vi "gRPC Server.vi"(8 "error in (no error)":errorcluster, 11 "CIFPlugin in":refnum<class "CAN_Writer_CANsub_Plugin.lvclass">) -> (0 "error out":errorcluster, 3 "CIFPlugin out":refnum<class "CAN_Writer_CANsub_Plugin.lvclass">)   [LabVIEW 2021, in "CAN_Writer_CANsub_Plugin.lvclass"]
uses:
  CAN_Writer_CANsub_Plugin.lvclass
  CAN_Writer_CANsub_Plugin.lvclass/CAN_Writer_CANsub_Plugin.ctl
  <vilib>/CIF Foundation/CIF Core/CIFCore/Class/CIFCorePlugin.lvclass
  Grpc/CanWriterCansub_server/RPC Messages/cif_common_Status.ctl
  Grpc/CanWriterCansub_server/CanWriterCansub_server.lvlib
  Grpc/CanWriterCansub_server/RPC Messages/cif_can_writer_cansub_Statistics.ctl
  Grpc/CanWriterCansub_server/RPC Service/CanWriterCansub/CanWriterCansub.lvclass
  <vilib>/CIF Foundation/CIF XNET CAN RW/XNET CAN RW.lvclass
  <vilib>/xnet/xnet.llb/XNET Blink Modifier.ctl
  Common/CAN_Writer_CANsub_Common.lvlib
  Common/Typedef/Errors.ctl
  Grpc/CanWriterCansub_server/RPC Messages/cif_can_writer_cansub_CommState.ctl
  Grpc/CanWriterCansub_server/RPC Messages/cif_can_writer_cansub_LastError.ctl
  Grpc/CanWriterCansub_server/RPC Messages/cif_can_writer_cansub_GetCANStatusResponse.ctl
  Grpc/CanWriterCansub_server/RPC Messages/cif_can_writer_cansub_CansubDevice.ctl
  Grpc/CanWriterCansub_server/RPC Messages/cif_can_writer_cansub_CansubDevices.ctl
  C:/Program Files/National Instruments/LabVIEW 2021/vi.lib/CIF Foundation/CIF Core/CIFCore/Class/CIFCorePlugin.lvclass
  D:/dev/Plugins/CAN_Writer_CANsub/Class/CAN_Writer_CANsub_Plugin.lvclass
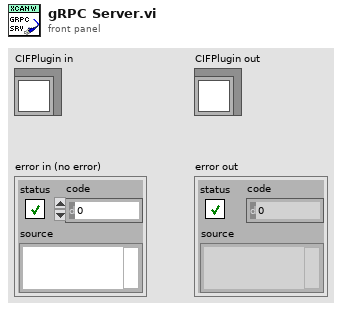
[diagram p1: front panel]
types:
  T1 = typedef "CanWriterCansub_server.lvlib/cif_can_writer_cansub_CansubDevices.ctl" = cluster{"devices":T2[]}
  T2 = typedef "CanWriterCansub_server.lvlib/cif_can_writer_cansub_CansubDevice.ctl" = cluster{"interface":string, "slot":u32, "device_id":string}
  T3 = typedef "CanWriterCansub_server.lvlib/cif_can_writer_cansub_GetCANStatusResponse.ctl" = cluster{"comm_state":T4, "last_error":T5, "rx_error_ctr":u32, "tx_error_crt":u32}
  T4 = typedef "CanWriterCansub_server.lvlib/cif_can_writer_cansub_CommState.ctl" = enum32{"COMMSTATE_ERROR_ACTIVE", "COMMSTATE_ERROR_PASSIVE", "COMMSTATE_BUS_OFF"}
  T5 = typedef "CanWriterCansub_server.lvlib/cif_can_writer_cansub_LastError.ctl" = enum32{"LASTERROR_NONE", "LASTERROR_STUFF", "LASTERROR_FORM", "LASTERROR_ACK", "LASTERROR_BIT1", "LASTERROR_BIT0", "LASTERROR_CRC", "LASTERROR_UNKNOWN"}
  T6 = typedef "CanWriterCansub_server.lvlib/cif_common_Status.ctl" = cluster{"code":i32, "message":string}
  T7 = typedef "CAN_Writer_CANsub_Common.lvlib/Errors.ctl" = enum16{"Invalid Interface"}
  T8 = typedef "XNET CAN RW.lvclass/XNET Devices.ctl" = cluster{"ID":string, "Slot":u32, "Interfaces":string[]}
  T9 = typedef "grpc-lvsupport-release.lvlib/grpcId.ctl" = u64
  T10 = typedef "CanWriterCansub_server.lvlib/cif_can_writer_cansub_CanMessage.ctl" = cluster{"can_message":u8[]}
  T11 = typedef "CanWriterCansub_server.lvlib/cif_can_writer_cansub_RefreshDevices.ctl" = cluster{"refresh_device_list":bool}
  T12 = typedef "CanWriterCansub_server.lvlib/cif_can_writer_cansub_Statistics.ctl" = cluster{"iterations":u64, "fifo_read_timeouts":u64, "write_frames":u64, "filtered_frames":u64, "fifo_drops":u64, "ack_errors":u64}
  T13 = typedef "CAN_RW_CORE.lvclass/Communication State.ctl" = enum16{"Error Active", "Error Passive", "Bus Off"}
  T14 = typedef "CAN_RW_CORE.lvclass/Last Error.ctl" = enum16{"None", "Stuff", "Form", "Ack", "Bit1", "Bit0", "CRC", "Unknown"}
  T15 = typedef "XNET Blink Modifier.ctl" = u32
  T16 = typedef "CanWriterCansub_server.lvlib/cif_can_writer_cansub_InterfaceBlink.ctl" = cluster{"blink":bool}
  T17 = typedef "CAN_Writer_CANsub_Common.lvlib/Configuration.ctl" = cluster{"Common":T18, "TX Interface":string, "Port Configuration":T20, "Filter":T23, "Wake Offset (us)":i64, "One Shot":bool}
  T18 = typedef "CIFCoreCommon.lvlib/Common Plugin Configuration.ctl" = cluster{"Period (s)":dbl, "Offset (us)":i32, "Priority":i32, "Processor":i32, "External Clock":T19}
  T19 = typedef "CIFCoreCommon.lvlib/External Clock Config.ctl" = cluster{"ClockID":u8, "Clock Name":string, "Publish Clock":bool, "Convert Data Timestamps":bool, "Plugin Timing Source":bool}
  T20 = typedef "CAN_RW_CORE.lvclass/CAN Port Configuration.ctl" = cluster{"Mode":T21, "Baud Rate":u64, "Temination On":bool, "Subordinate":bool, "Echo TX":bool, "FD Config":T22}
  T21 = typedef "CAN_RW_CORE.lvclass/CAN Mode.ctl" = enum16{"CAN 2.0", "CAN FD"}
  T22 = typedef "CAN_RW_CORE.lvclass/FD Config.ctl" = cluster{"FD Baud Rate":u64, "ISO Mode":bool, "BRS Enabled":bool}
  T23 = typedef "CAN_RW_CORE.lvclass/CAN Filter.ctl" = cluster{"Allow List (ID)":u32[], "Deny List (ID)":u32[]}
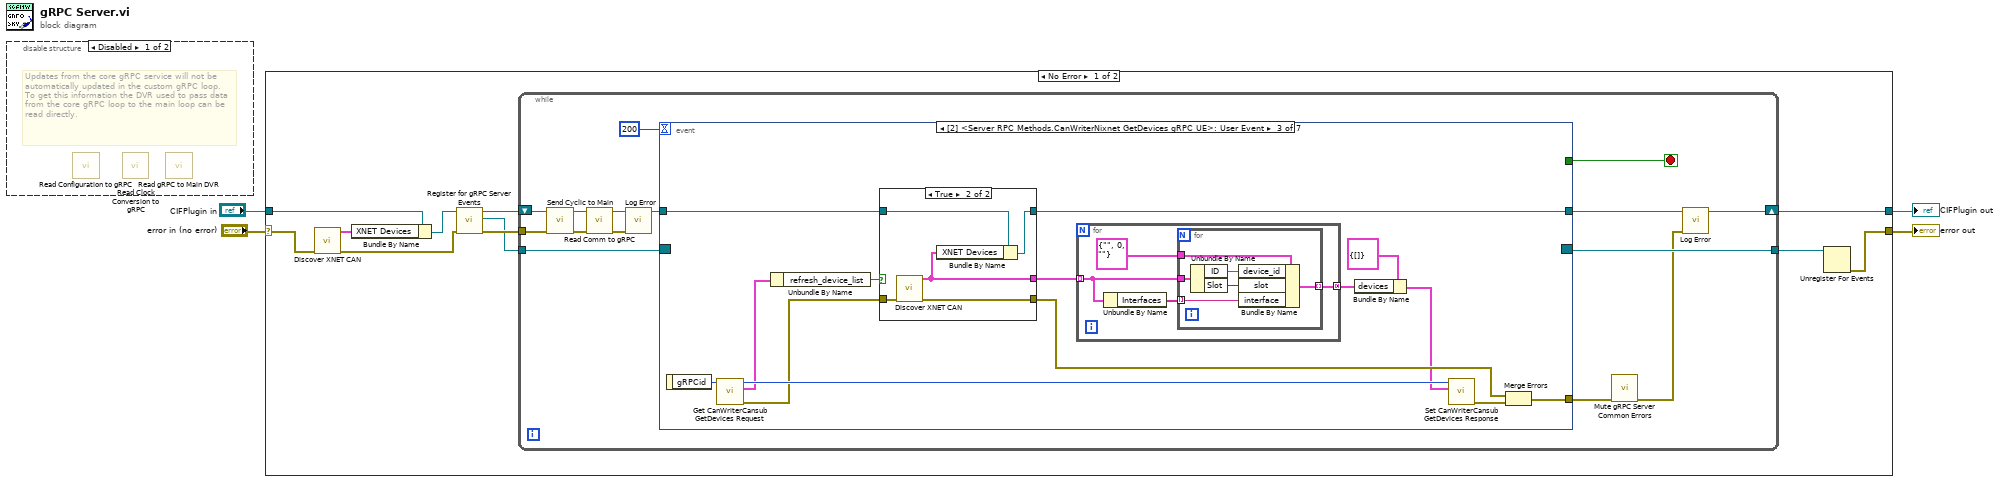
[diagram p0: block diagram]
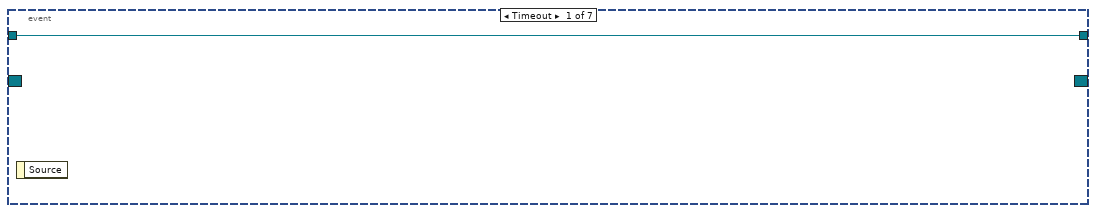
[diagram p3: hidden frame]
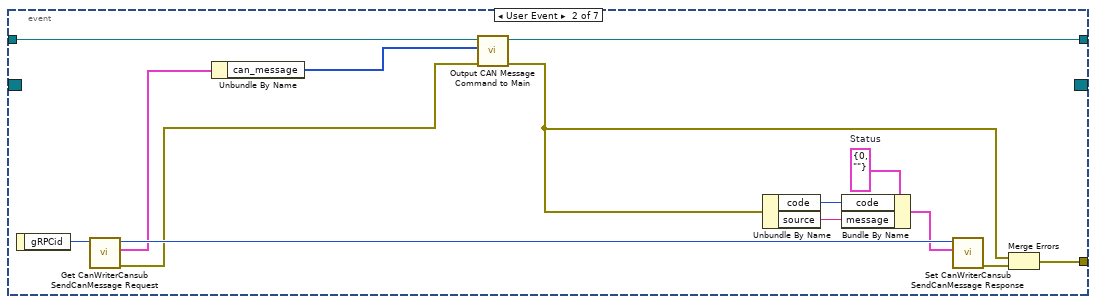
[diagram p4: hidden frame]
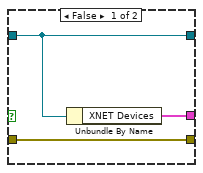
[diagram p5: hidden frame]
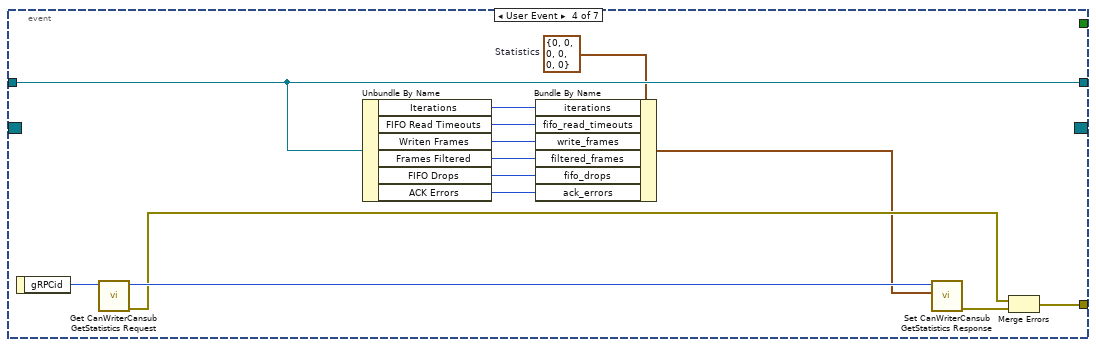
[diagram p6: hidden frame]
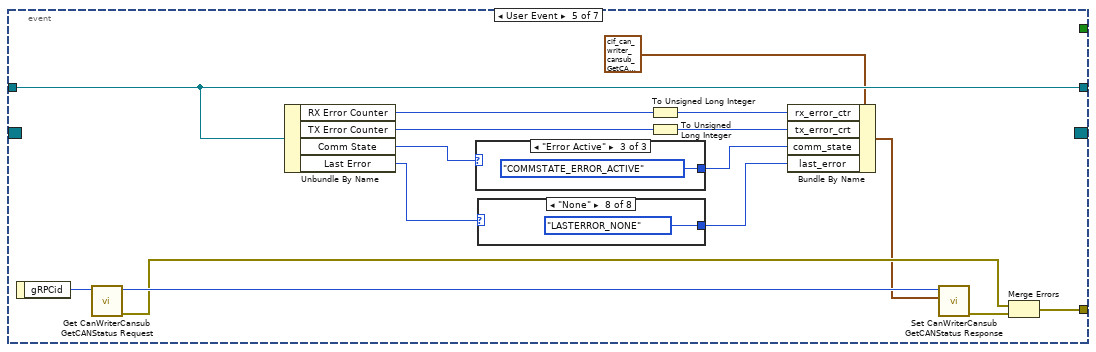
[diagram p7: hidden frame]
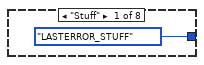
[diagram p8: hidden frame]
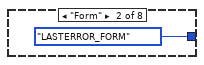
[diagram p9: hidden frame]
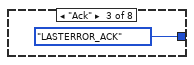
[diagram p10: hidden frame]
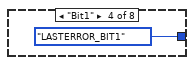
[diagram p11: hidden frame]
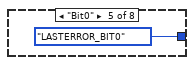
[diagram p12: hidden frame]
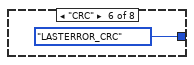
[diagram p13: hidden frame]
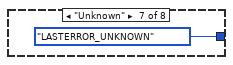
[diagram p14: hidden frame]
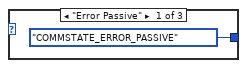
[diagram p15: hidden frame]
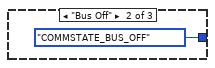
[diagram p16: hidden frame]
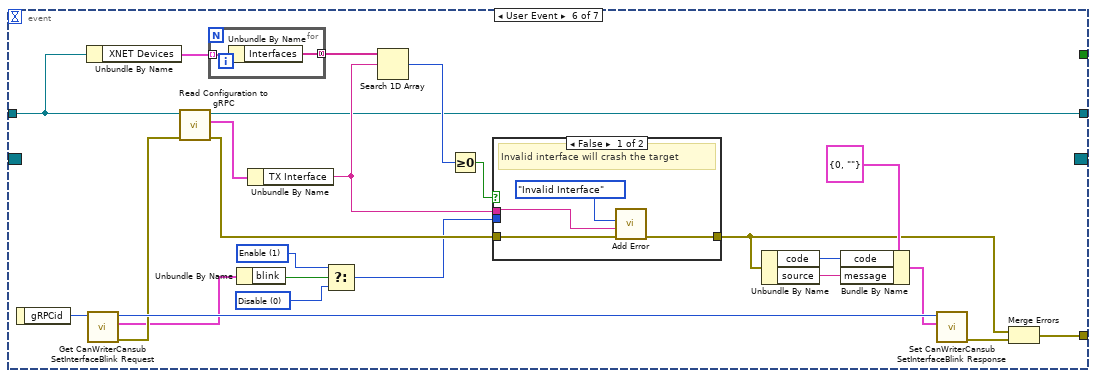
[diagram p17: hidden frame]
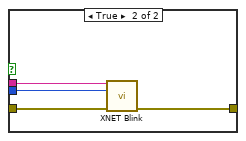
[diagram p18: hidden frame]
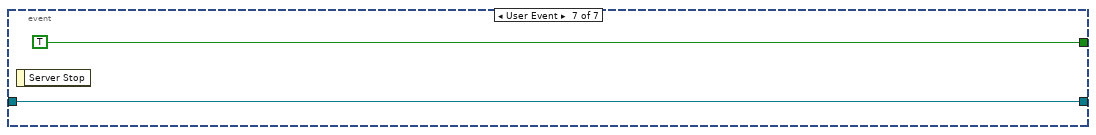
[diagram p19: hidden frame]
diagram:
  n1 = disable-structure shown="Disabled" {
    frame Disabled {
      # "Updates from the core gRPC service will not be automatically updated in the custom gRPC loop.  To get this information the DVR used to pass data from the core gRPC loop to the main loop can be read directly."
      n2 = call "Read Configuration to gRPC.vi"() -> ()  [unwired: 9 in, 3 out]
      n3 = call <vilib>:"Read Clock Conversion to gRPC.vi"() -> ()  [unwired: 9 in, 3 out]
      n4 = call <vilib>:"Read gRPC to Main DVR.vi"() -> ()  [unwired: 9 in, 3 out]
    }
    frame Enabled {
    }
  }
  n5 = case shown="No Error" "error in (no error)" {
    selector: "error in (no error)" -> [w6 w155]
    tunnel: "CIFPlugin in" -> [w9 w156]
    tunnel: [w14 w156] -> w3
    tunnel: [w11 w155] -> w4
    frame No Error {
      n6 = call <vilib>:"Discover XNET CAN.vi"("error in (no error)"=w6) -> ("error out"=w5:errorcluster, "XNET Devices"=w7:T8[])  [unwired: 9 in]
      n7 = Bundle By Name(cluster=w9, "XNET Devices"=w7) -> (w8:refnum<class "CAN_Writer_CANsub_Plugin.lvclass">)
      n8 = call "Register for gRPC Server Events.vi"("error in (no error)"=w5, "CIFPlugin in"=w8) -> ("error out"=w13:errorcluster, "Event Registration Refnum"=w10:refnum<event-registration>, "CIFPlugin out"=w12:refnum<class "CAN_Writer_CANsub_Plugin.lvclass">)  [unwired: 7 in]
      n9 = while {
        tunnel: w10 -> [w18]
        tunnel: w13 -> [w23]
        tunnel: [w28] -> w15
        shift-right: [w26] -> w14
        shift-left: w12 -> [w24]
        stop <- w29 stop-if-true
        n10 = call "Send Cyclic to Main.vi"("error in (no error)"=w23, "CIFPlugin in"=w24) -> ("error out"=w21:errorcluster, "CIFPlugin out"=w22:refnum<class "CAN_Writer_CANsub_Plugin.lvclass">)  [unwired: 8 in]
        n11 = call "Read Comm to gRPC.vi"("error in (no error)"=w21, "CIFPlugin in"=w22) -> ("error out"=w19:errorcluster, "CIFPlugin out"=w20:refnum<class "CAN_Writer_CANsub_Plugin.lvclass">)  [unwired: 8 in]
        n12 = call <vilib>:"Log Error.vi"("error in (no error)"=w19, "CIFCorePlugin in"=w20) -> ("CIFCorePlugin out"=w25:refnum<class "CAN_Writer_CANsub_Plugin.lvclass">)  [unwired: 8 in, 1 out]
        n13 = event shown="[2] <Server RPC Methods.CanWriterNixnet GetDevices gRPC UE>: User Event" {
          selector: w18 -> [_ _ _ _ _ _ _]
          dyn-events: [_ _ _ _ _ _ _] -> w28
          timeout: 200 -> [_ _ _ _ _ _ _]
          tunnel: w25 -> [w31 w36 w50 w90 w106 w119 w153]
          tunnel: [_ w43 w59 w91 w107 w142 _] -> w17
          tunnel: [w31 w32 w49 w90 w106 w125 w153] -> w27
          tunnel: [_ _ _ _ _ _ TRUE] -> w29
          event Timeout {
            n14 = event-data() -> ()  [unwired: 1 in, 1 out]
          }
          event User Event {
            w42 = T6 {"code"=0, "message"=""}  # Status
            n15 = event-data() -> ("gRPCid"=w40:T9)  [unwired: 1 in]
            n16 = call "Get CanWriterCansub SendCanMessage Request.vi"("gRPCid"=w40) -> ("error out"=w34:errorcluster, "Message Data"=w38:T10, "gRPCid out"=w41:T9)  [unwired: 8 in]
            n17 = Unbundle By Name(w38) -> ("can_message"=w35:u8[])
            n18 = call "Output CAN Message Command to Main.vi"("error in (no error)"=w34, "Output Message"=w35, "CIFPlugin in"=w36) -> ("error out"=w33:errorcluster, "CIFPlugin out"=w32:refnum<class "CAN_Writer_CANsub_Plugin.lvclass">)  [unwired: 7 in]
            n19 = Unbundle By Name(w33) -> ("code"=w45:i32, "source"=w44:string)
            n20 = Bundle By Name(cluster=w42, "code"=w45, "message"=w44) -> (w37:T6)
            n21 = call "Set CanWriterCansub SendCanMessage Response.vi"("Message Data"=w37, "gRPCid in"=w41) -> ("error out"=w39:errorcluster)  [unwired: 9 in]
            n22 = Merge Errors(w33, w39) -> (w43:errorcluster)
          }
          event User Event {
            n23 = event-data() -> ("gRPCid"=w57:T9)  [unwired: 1 in]
            n24 = call "Get CanWriterCansub GetDevices Request.vi"("gRPCid"=w57) -> ("error out"=w51:errorcluster, "Message Data"=w52:T11, "gRPCid out"=w58:T9)  [unwired: 8 in]
            n25 = Unbundle By Name(w52) -> ("refresh_device_list"=w53:bool)
            n26 = case shown="True" w53 {
              tunnel: w50 -> [w71 w77]
              tunnel: w51 -> [w72 w76]
              tunnel: [w72 w75] -> w48
              tunnel: [w71 w74] -> w49
              tunnel: [w70 w73] -> w55
              frame False {
                n27 = Unbundle By Name(w71) -> ("XNET Devices"=w70:T8[])
              }
              frame True {
                n28 = call <vilib>:"Discover XNET CAN.vi"("error in (no error)"=w76) -> ("error out"=w75:errorcluster, "XNET Devices"=w73:T8[])  [unwired: 9 in]
                n29 = Bundle By Name(cluster=w77, "XNET Devices"=w73) -> (w74:refnum<class "CAN_Writer_CANsub_Plugin.lvclass">)
              }
            }
            n30 = for {
              tunnel: w55 -> [w62] mode=indexing
              tunnel: [w61] -> w54 mode=concatenating
              n31 = Unbundle By Name(w62) -> ("Interfaces"=w63:string[])
              n32 = for {
                tunnel: w63 -> [w66] mode=indexing
                tunnel: w62 -> [w69]
                tunnel: T2 {"interface"="", "slot"=0, "device_id"=""} ("cif_can_writer_cansub_CansubDevice") -> [w68]
                tunnel: [w64] -> w61 mode=indexing
                n33 = Unbundle By Name(w69) -> ("ID"=w67:string, "Slot"=w65:u32)
                n34 = Bundle By Name(cluster=w68, "device_id"=w67, "slot"=w65, "interface"=w66) -> (w64:T2)
              }
            }
            n35 = Bundle By Name(cluster=T1 {"devices"=[]} ("Message Data"), "devices"=w54) -> (w47:T1)
            n36 = call "Set CanWriterCansub GetDevices Response.vi"("Message Data"=w47, "gRPCid in"=w58) -> ("error out"=w56:errorcluster)  [unwired: 9 in]
            n37 = Merge Errors(w48, w56) -> (w59:errorcluster)
          }
          event User Event {
            w84 = T12 {"iterations"=0, "fifo_read_timeouts"=0, "write_frames"=0, "filtered_frames"=0, "fifo_drops"=0, "ack_errors"=0}  # Statistics
            n38 = event-data() -> ("gRPCid"=w80:T9)  [unwired: 1 in]
            n39 = call "Get CanWriterCansub GetStatistics Request.vi"("gRPCid"=w80) -> ("error out"=w86:errorcluster, "gRPCid out"=w88:T9)  [unwired: 8 in, 1 out]
            n40 = Unbundle By Name(w90) -> ("Iterations"=w89:u64, "FIFO Read Timeouts"=w81:u64, "Writen Frames"=w82:u64, "Frames Filtered"=w83:u64, "FIFO Drops"=w79:u64, "ACK Errors"=w78:u64)
            n41 = Bundle By Name(cluster=w84, "iterations"=w89, "fifo_read_timeouts"=w81, "write_frames"=w82, "filtered_frames"=w83, "fifo_drops"=w79, "ack_errors"=w78) -> (w85:T12)
            n42 = call "Set CanWriterCansub GetStatistics Response.vi"("Message Data"=w85, "gRPCid in"=w88) -> ("error out"=w87:errorcluster)  [unwired: 9 in]
            n43 = Merge Errors(w86, w87) -> (w91:errorcluster)
          }
          event User Event {
            n44 = event-data() -> ("gRPCid"=w102:T9)  [unwired: 1 in]
            n45 = call "Get CanWriterCansub GetCANStatus Request.vi"("gRPCid"=w102) -> ("error out"=w101:errorcluster, "gRPCid out"=w103:T9)  [unwired: 8 in, 1 out]
            n46 = Unbundle By Name(w106) -> ("RX Error Counter"=w105:u8, "TX Error Counter"=w104:u8, "Comm State"=w95:T13, "Last Error"=w93:T14)
            n47 = case shown="\"Error Active\"" w95 {
              tunnel: [cif_can_writer_cansub_CommState."COMMSTATE_ERROR_PASSIVE" ("comm_state") cif_can_writer_cansub_CommState."COMMSTATE_BUS_OFF" ("comm_state") cif_can_writer_cansub_CommState."COMMSTATE_ERROR_ACTIVE" ("comm_state")] -> w94
              frame "Error Passive" {
              }
              frame "Bus Off" {
              }
              frame "Error Active" {
              }
            }
            n48 = case shown="\"None\"" w93 {
              tunnel: [cif_can_writer_cansub_LastError."LASTERROR_STUFF" ("last_error") cif_can_writer_cansub_LastError."LASTERROR_FORM" ("last_error") cif_can_writer_cansub_LastError."LASTERROR_ACK" ("last_error") cif_can_writer_cansub_LastError."LASTERROR_BIT1" ("last_error") cif_can_writer_cansub_LastError."LASTERROR_BIT0" ("last_error") cif_can_writer_cansub_LastError."LASTERROR_CRC" ("last_error") cif_can_writer_cansub_LastError."LASTERROR_UNKNOWN" ("last_error") cif_can_writer_cansub_LastError."LASTERROR_NONE" ("last_error")] -> w92
              frame "Stuff" {
              }
              frame "Form" {
              }
              frame "Ack" {
              }
              frame "Bit1" {
              }
              frame "Bit0" {
              }
              frame "CRC" {
              }
              frame "Unknown" {
              }
              frame "None" {
              }
            }
            n49 = To Unsigned Long Integer(number=w105) -> (unsigned 32bit integer=w97:u32)
            n50 = To Unsigned Long Integer(number=w104) -> (unsigned 32bit integer=w98:u32)
            n51 = Bundle By Name(cluster=T3 {"comm_state"=enum."COMMSTATE_ERROR_ACTIVE", "last_error"=enum."LASTERROR_NONE", "rx_error_ctr"=0, "tx_error_crt"=0} ("Message Data"), "rx_error_ctr"=w97, "tx_error_crt"=w98, "comm_state"=w94, "last_error"=w92) -> (w96:T3)
            n52 = call "Set CanWriterCansub GetCANStatus Response.vi"("Message Data"=w96, "gRPCid in"=w103) -> ("error out"=w100:errorcluster)  [unwired: 9 in]
            n53 = Merge Errors(w101, w100) -> (w107:errorcluster)
          }
          event User Event {
            w126 = T15 1 items=["Disable", "Enable"] ("modifier")
            w127 = T15 0 items=["Disable", "Enable"] ("modifier")
            n54 = event-data() -> ("gRPCid"=w141:T9)  [unwired: 1 in]
            n55 = Unbundle By Name(w119) -> ("XNET Devices"=w132:T8[])
            n56 = call "Get CanWriterCansub SetInterfaceBlink Request.vi"("gRPCid"=w141) -> ("error out"=w122:errorcluster, "Message Data"=w120:T16, "gRPCid out"=w140:T9)  [unwired: 8 in]
            n57 = call "Read Configuration to gRPC.vi"("error in (no error)"=w122, "CIFPlugin in"=w119) -> ("error out"=w138:errorcluster, "Configuration"=w137:T17, "CIFPlugin out"=w125:refnum<class "CAN_Writer_CANsub_Plugin.lvclass">)  [unwired: 7 in]
            n58 = for {
              tunnel: w132 -> [w144] mode=indexing
              tunnel: [w143] -> w133 mode=concatenating
              n59 = Unbundle By Name(w144) -> ("Interfaces"=w143:string[])
            }
            n60 = Unbundle By Name(w120) -> ("blink"=w130:bool)
            n61 = Unbundle By Name(w137) -> ("TX Interface"=w134:string)
            n62 = Select(t=w126, s=w130, f=w127) -> (s? t:f=w131:T15)
            n63 = Search 1D Array(1D array=w133, element=w134) -> (index of element=w135:i32)  [unwired: 1 in]
            n64 = Greater Or Equal To 0?(x=w135) -> (x >= 0?=w136:bool)
            n65 = case shown="False" w136 {
              tunnel: w134 -> [w145 w152]
              tunnel: w138 -> [w148 w151]
              tunnel: [w147 w150] -> w121
              tunnel: w131 -> [_ w149]
              frame False {
                # "Invalid interface will crash the target"
                n66 = call "Add Error.vi"("error in (no error)"=w148, "String to Append"=w145, "Error"=Errors."Invalid Interface") -> ("error out"=w147:errorcluster)  [unwired: 8 in]
              }
              frame True {
                n67 = call <vilib>:"XNET Blink.vi"("interface in"=w152, "modifier"=w149, "error in (no error)"=w151) -> ("error out"=w150:errorcluster)  [unwired: 11 in, 1 out]
              }
            }
            n68 = Unbundle By Name(w121) -> ("code"=w128:i32, "source"=w129:string)
            n69 = Bundle By Name(cluster=T6 {"code"=0, "message"=""} ("Message Data"), "code"=w128, "message"=w129) -> (w123:T6)
            n70 = call "Set CanWriterCansub SetInterfaceBlink Response.vi"("Message Data"=w123, "gRPCid in"=w140) -> ("error out"=w139:errorcluster)  [unwired: 9 in]
            n71 = Merge Errors(w121, w139) -> (w142:errorcluster)
          }
          event User Event {
            n72 = event-data() -> ()  [unwired: 1 in, 1 out]
          }
        }
        n73 = call <vilib>:"Mute gRPC Server Common Errors.vi"("error in (no error)"=w17) -> ("error out"=w16:errorcluster)  [unwired: 10 in]
        n74 = call <vilib>:"Log Error.vi"("error in (no error)"=w16, "CIFCorePlugin in"=w27) -> ("CIFCorePlugin out"=w26:refnum<class "CAN_Writer_CANsub_Plugin.lvclass">)  [unwired: 8 in, 1 out]
      }
      n75 = Unregister For Events(event registration refnum=w15) -> (error out=w11:errorcluster)  [unwired: 1 in]
    }
    frame Error {
    }
  }
  "error out" <- w4
  "CIFPlugin out" <- w3
